vi "Moviment jugador.vi"(8 "error in (no error)":errorcluster, 9 "LINX Resource in":T1, 10 "y jugador":dbl, 11 "x jugador":dbl) -> (0 "error out":errorcluster, 1 "y final jugador":dbl, 2 "x final jugador":dbl, 3 "Cluster":cluster{dbl[], dbl[]}, 5 "LINX Resource out":T1)   [LabVIEW 2023]
uses:
  <vilib>/MakerHub/LINX/Private/Type Defs/LINX Ref.ctl
  <vilib>/MakerHub/LINX/Private/Type Defs/Platform.ctl
  <vilib>/MakerHub/LINX/Private/Type Defs/Interface.ctl
  <vilib>/MakerHub/LINX/Private/Device/Type Defs/LINX Device Config.ctl
  <vilib>/MakerHub/LINX/Private/Device/Type Defs/TCP Config.ctl
  <vilib>/MakerHub/LINX/Private/Device/Type Defs/Channels.ctl
  <vilib>/MakerHub/LINX/Public/Peripherals/Analog/Analog Read N Chans.vi
  <vilib>/MakerHub/LINX/Private/Local IO/LinxAnalogRead.vi
  <vilib>/MakerHub/LINX/Public/Utilities/Check Channel.vi
  <vilib>/MakerHub/LINX/Private/Utilties/Generate Error.vi
  <vilib>/MakerHub/LINX/LMH-LINX.lvlib
  <vilib>/MakerHub/LINX/Private/Device/Device.lvlib
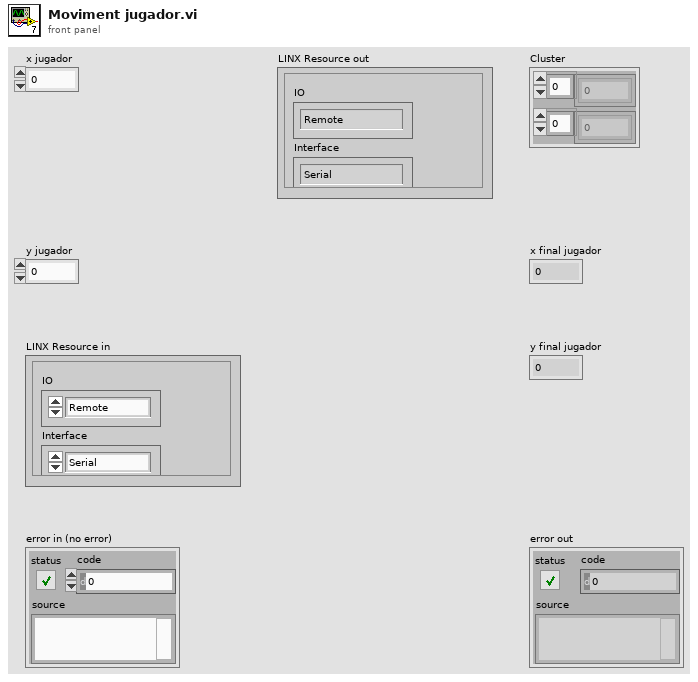
[diagram p1: front panel]
types:
  T1 = typedef "LMH-LINX.lvlib/LINX Ref.ctl" = cluster{"IO":T2, "Interface":T3, "LINX Device Config":T4}
  T2 = typedef "LMH-LINX.lvlib/Platform.ctl" = enum16{"Remote", "Local"}
  T3 = typedef "LMH-LINX.lvlib/Interface.ctl" = enum16{"Serial", "TCP"}
  T4 = typedef "LMH-LINX.lvlib/Device.lvlib/LINX Device Config.ctl" = cluster{"Interface":T3, "COM Port":refnum<visa-resource-name>, "TCP Configuration":T5, "Device Family":u8, "Device ID":u8, "Device Name":string, "TCP Ref":refnum<k5>, "Channels":T6}
  T5 = typedef "LMH-LINX.lvlib/Device.lvlib/TCP Config.ctl" = cluster{"IP Address":string, "Port":u16}
  T6 = typedef "LMH-LINX.lvlib/Channels.ctl" = cluster{"DI":u8[], "DO":u8[], "AI":u8[], "AO":u8[], "PWM":u8[], "QE":u8[], "UART":u8[], "I2C 2":u8[], "SPI":u8[], "CAN":u8[], "Servo":u8[], "AI Ref (V)":dbl, "AI Resolution (Bits)":u8, "AO Ref (V)":dbl, "AO Resolution (Bits)":u8}
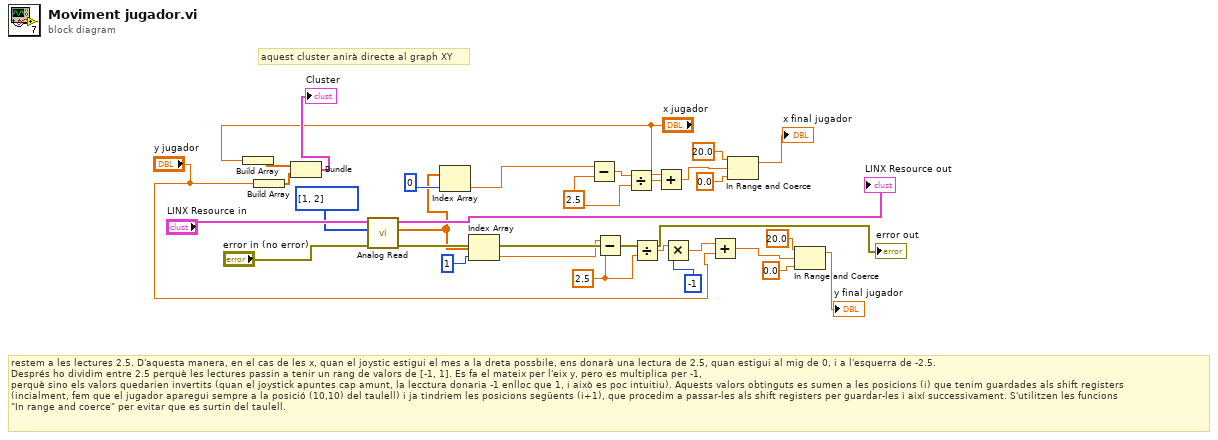
[diagram p0: block diagram]
diagram:
  w10 = 2.5
  w9 = 2.5
  # "restem a les lectures 2.5. D'aquesta manera, en el cas de les x, quan el joystic estigui el mes a la dreta possbile, ens donarà una lectura de 2.5, quan estigui al mig de 0, i a l'esquerra de -2.5. \nDesprés ho dividim entre 2.5 perquè les lectures passin a tenir un rang de valors de [-1, 1]. Es fa el mateix per l'eix y, pero es multiplica per -1, \nperquè sino els valors quedarien invertits (quan el joystick apuntes cap amunt, la lecctura donaria -1 enlloc que 1, i això es poc intuitiu). Aquests valors obtinguts es sumen a les posicions (i) que tenim guardades als shift registers \n(incialment, fem que el jugador aparegui sempre a la posició (10,10) del taulell) i ja tindriem les posicions següents (i+1), que procedim a passar-les als shift registers per guardar-les i així successivament. S'utilitzen les funcions \n\"In range and coerce\" per evitar que es surtin del taulell."
  # "aquest cluster anirà directe al graph XY"
  n1 = Build Array("x jugador") -> (w3:dbl[])
  n2 = Build Array("y jugador") -> (w13:dbl[])
  n3 = Bundle(w3, w13) -> (→"Cluster":cluster{dbl[], dbl[]})  [unwired: 1 in]
  n4 = call-poly <vilib>:"Analog Read.vi"("Error In"="error in (no error)", "AI Channel(s)"=u8[] [1, 2], "LINX Resource"="LINX Resource in") -> ("Error Out"=→"error out":errorcluster, "Voltages"=w5:dbl[], "LINX Resource"=→"LINX Resource out":T1)  [unwired: 5 in, 1 out]
  n5 = Index Array(array=w5, index=0) -> (element=w7:dbl)
  n6 = Index Array(array=w5, index=1) -> (element=w8:dbl)
  n7 = Subtract(x=w7, y=w9) -> (x-y=w2:dbl)
  n8 = Subtract(x=w8, y=w10) -> (x-y=w15:dbl)
  n9 = Divide(x=w2, y=w9) -> (x/y=w11:dbl)
  n10 = Divide(x=w15, y=w10) -> (x/y=w16:dbl)
  n11 = Add(x="x jugador", y=w11) -> (x+y=w23:dbl)
  n12 = Multiply(x=w16, y=-1) -> (x*y=w17:dbl)
  n13 = Add(x=w17, y="y jugador") -> (x+y=w27:dbl)
  n14 = In Range and Coerce(upper limit=20.0, x=w23, lower limit=0.0) -> (coerced(x)=→"x final jugador":dbl)  [unwired: 1 out]
  n15 = In Range and Coerce(upper limit=20.0, x=w27, lower limit=0.0) -> (coerced(x)=→"y final jugador":dbl)  [unwired: 1 out]
